vi "RT.vi"() -> ()   [LabVIEW 2025]
uses:
  Cluster_TH.ctl
  <vilib>/FPGAPlugInAG/myRIO-1900/niLvFpga_Open_myRIO-1900.vi
  <vilib>/rvi/interface/common/dynamic/niFpgaDynamicAddResources.vi
  <vilib>/FPGAPlugInAG/Dynamic/niLvFpga_Reset_Dynamic.vi
  <vilib>/Utility/error.llb/Error Cluster From Error Code.vi
  <vilib>/rvi/errors/niLvFpgaAdjustHostInterfaceError.vi
  <vilib>/rvi/interface/common/niFpgaWaitOnOcc.vi
  <vilib>/FPGAPlugInAG/Dynamic/niLvFpga_Run_Dynamic.vi
  <vilib>/FPGAPlugInAG/Dynamic/niLvFpga_Close_Dynamic.vi
  <vilib>/rvi/interface/nirviOpenFPGA/nirviOpenFPGA.xnode
  FPGA Bitfiles/michalwojna_FPGATarget_FPGA_Jo2F8lJHhgk.lvbitx
  FPGA.vi
  <vilib>/rvi/interface/nirviMethod/nirviMethod.xnode
  <vilib>/rvi/interface/nirviReadWriteControl/nirviReadWriteControl.xnode
  <vilib>/rvi/interface/nirviCloseFPGA/nirviCloseFPGA.xnode
  <vilib>/rvi/errors/niLvFpgaMergeErrorWithErrorCode.vi
  NiFpgaLv.dll
  <vilib>/rvi/interface/Simulation/niFpgaSimulationCallBeginRW.vi
  <vilib>/FPGAPlugInAG/Dynamic/niLvFpga_ConfigureFifo_Dynamic.vi
  <vilib>/FPGAPlugInAG/Dynamic/niLvFpga_ReadFifo_Dynamic.vi
panel:
  in  "Z_TH":i16
  in  "Y_TH":i16
  in  "X_TH":i16
  in  "Thresholds":T1={"X_TH"=400, "Y_TH"=400, "Z_TH"=400}
  out "X":i16[][](graph)
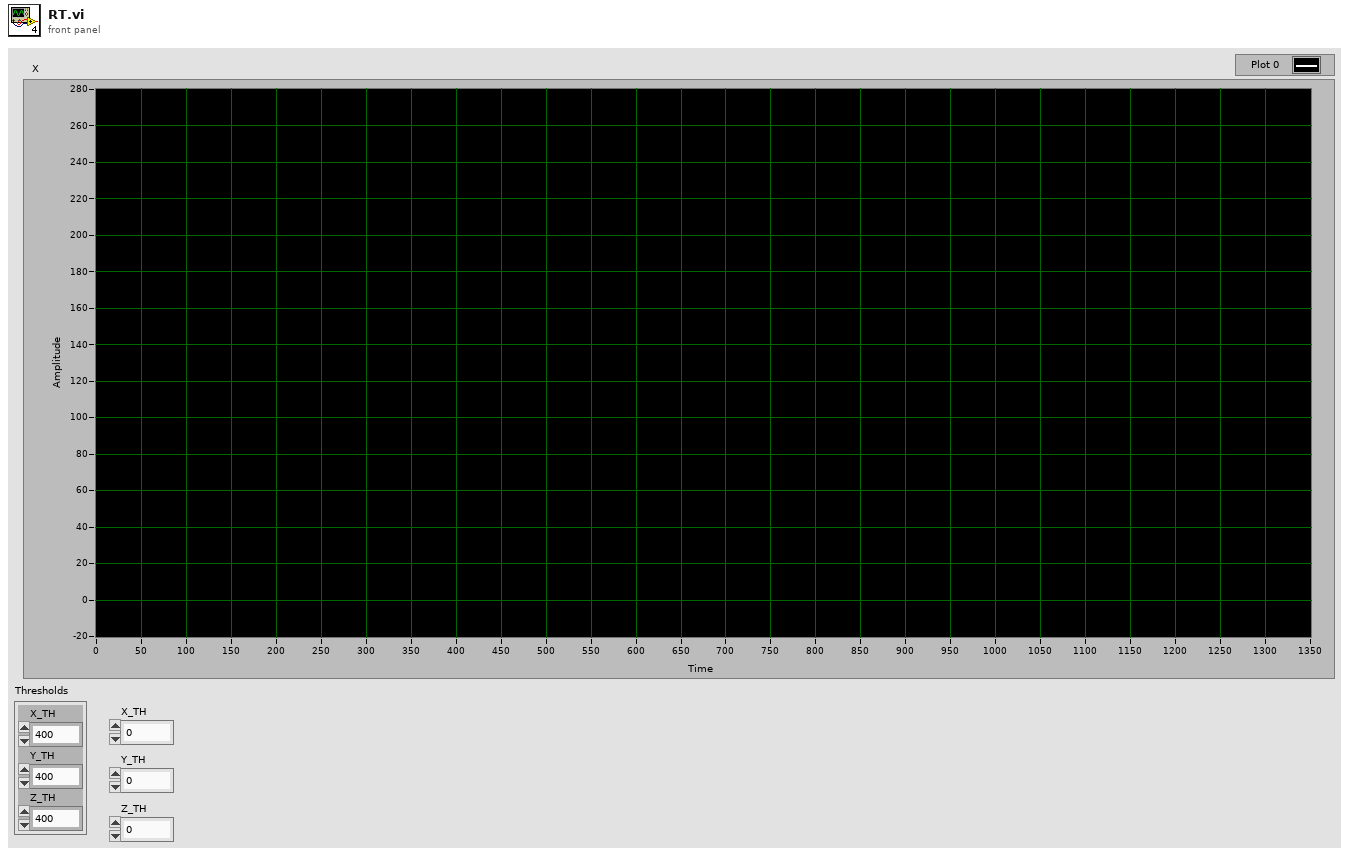
[diagram p1: front panel]
types:
  T1 = typedef "Cluster_TH.ctl" = cluster{"X_TH":i16, "Y_TH":i16, "Z_TH":i16}
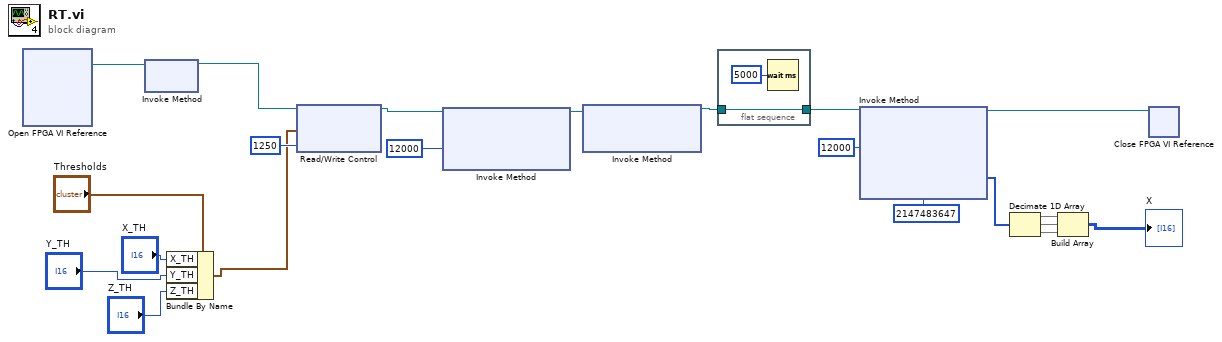
[diagram p0: block diagram]
diagram:
  n1 = xnode "Open FPGA VI Reference"() -> ("FPGA VI Reference Out"=w2:refnum<k20>)  [unwired: 2 in, 1 out]
  n2 = xnode "Invoke Method"("FPGA VI Reference In"=w2) -> ("FPGA VI Reference Out"=w1:refnum<k20>)  [unwired: 1 in, 1 out]
  n3 = Bundle By Name(cluster="Thresholds", "X_TH"="X_TH", "Y_TH"="Y_TH", "Z_TH"="Z_TH") -> (w11:T1)
  n4 = xnode "Read/Write Control"("FPGA VI Reference In"=w1, "THs"=w11, "Count(uSec)"=u32 1250) -> ("FPGA VI Reference Out"=w19:refnum<k20>)  [unwired: 1 in, 1 out]
  n5 = xnode "Invoke Method"("FPGA VI Reference In"=w19, "Requested Depth"=u32 12000) -> ("FPGA VI Reference Out"=w21:refnum<k20>)  [unwired: 1 in, 2 out]
  n6 = xnode "Invoke Method"("FPGA VI Reference In"=w21) -> ("FPGA VI Reference Out"=w17:refnum<k20>)  [unwired: 2 in, 1 out]
  n7 = flat-sequence {
    tunnel: [w22] -> w16
    tunnel: w17 -> [w22]
    frame #0 {
      n8 = Wait (ms)(milliseconds to wait=u32 5000) -> ()  [unwired: 1 out]
    }
  }
  n9 = xnode "Invoke Method"("FPGA VI Reference In"=w16, "Number of Elements"=u32 12000, "Timeout (ms)"=2147483647 ("Timeout")) -> ("FPGA VI Reference Out"=w15:refnum<k20>, "Data"=w7:i16[])  [unwired: 1 in, 2 out]
  n10 = Decimate 1D Array(w7) -> (w6:i16[], w5:i16[], w4:i16[])
  n11 = Build Array(w6, w5, w4) -> (→"X":i16[][])
  n12 = xnode "Close FPGA VI Reference"("FPGA VI Reference In"=w15) -> ()  [unwired: 1 in, 1 out]
